vi "Disable.vi"(8 "error in (no error)":errorcluster, 11 "logger name":string) -> (0 "error out":errorcluster)   [LabVIEW 2018, in "GLog.lvlib" / "Registry.lvlib"]
uses:
  Registry.lvlib
  Registry Actions.ctl
  dependencies/Utilities/Utilities.lvlib
panel:
  # "Connector Pane"
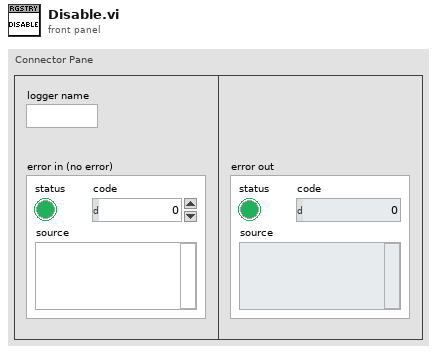
[diagram p1: front panel]
types:
  T1 = typedef "GLog.lvlib/Registry.lvlib/Registry Actions.ctl" = enum16{"Register", "Log", "Enable", "Enable All", "Disable", "Disable All", "Get Enable State", "Get Minimum Log Level", "Set Minimum Log Level", "Set All Minimum Log Level", "Get Logger Info", "Get All Logger Info", "List", "Unregister", "Unregister All", "Shutdown"}
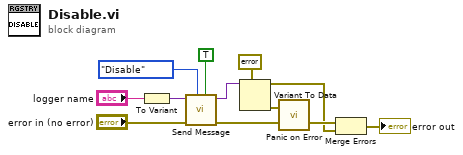
[diagram p0: block diagram]
diagram:
  n1 = To Variant(anything="logger name") -> (Variant=w9:variant)
  n2 = call "Send Message.vi"("return data? (F)"=TRUE, "action"=Registry_Actions."Disable", "error in (no error)"="error in (no error)", "send data"=w9) -> ("error out"=w10:errorcluster, "Variant"=w5:variant)  [unwired: 6 in]
  n3 = Variant To Data(type=errorcluster {"status"=FALSE, "code"=0, "source"=""} ("error in"), Variant=w5) -> (data=w2:errorcluster, error out=w4:errorcluster)  [unwired: 1 in]
  n4 = call "Panic on Error.vi"("error in (no error)"=w4) -> ()  [unwired: 3 in]
  n5 = Merge Errors(w10, w2) -> (→"error out":errorcluster)
